vi "_reorder tool entries.vi"(11 "Path Control":path[](array[path])) -> (2 "After":string[](array[string]), 3 "Path Control (dup)":path[](array[path]))   [LabVIEW 2017, in "CSM DebugTool Dialog.lvlib"]
uses:
  CSM DebugTool Dialog.lvlib
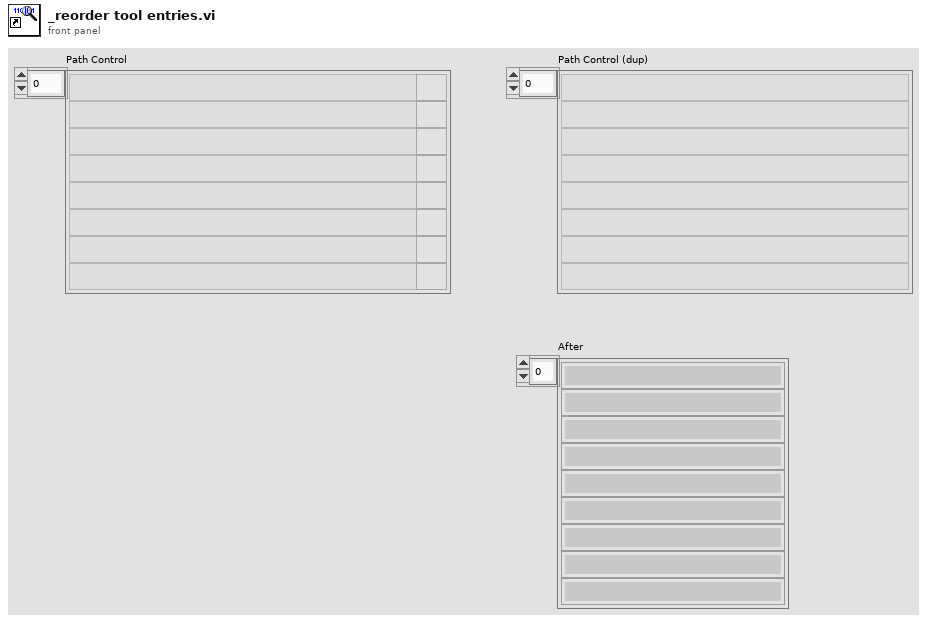
[diagram p1: front panel]
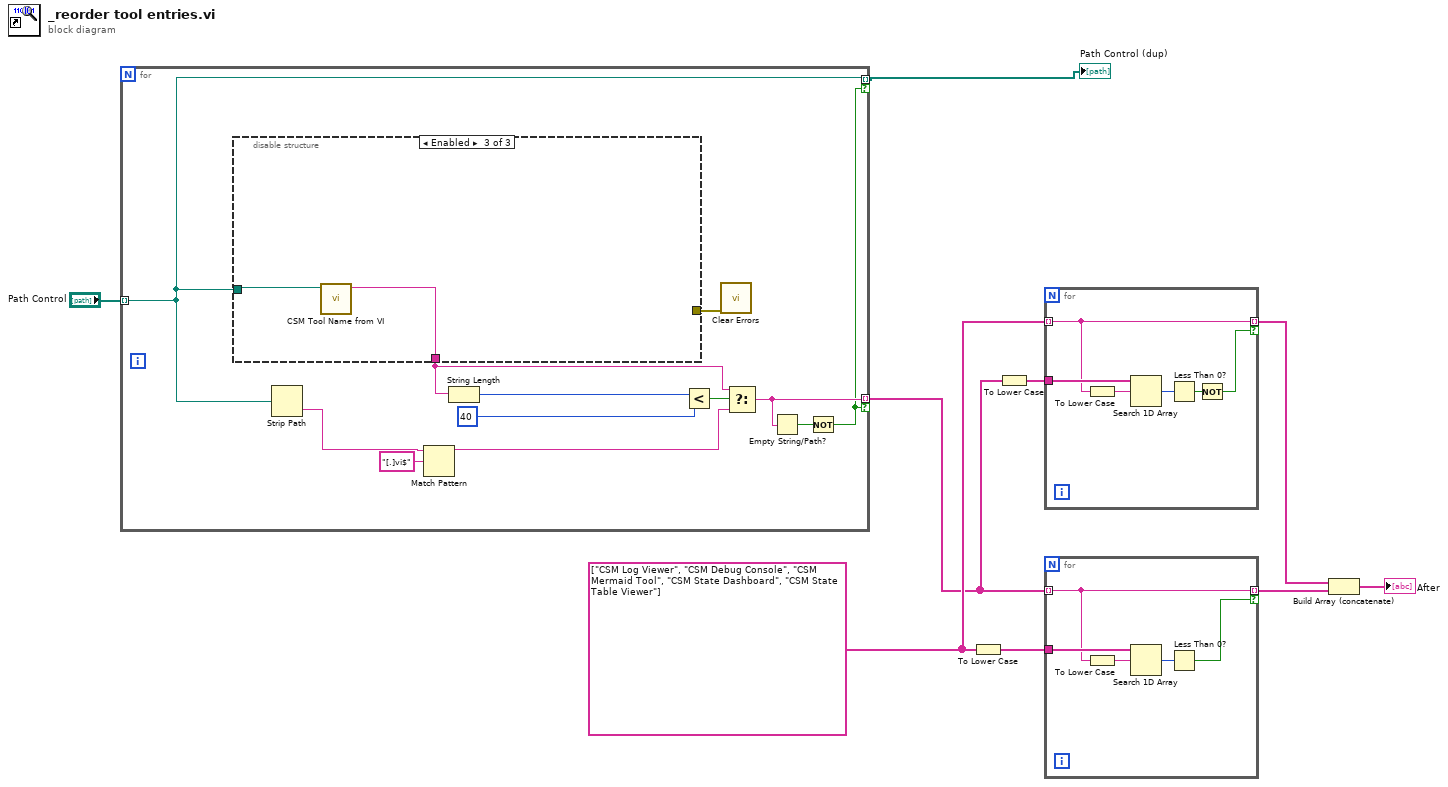
[diagram p0: block diagram]
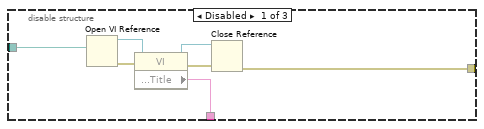
[diagram p2: hidden frame]
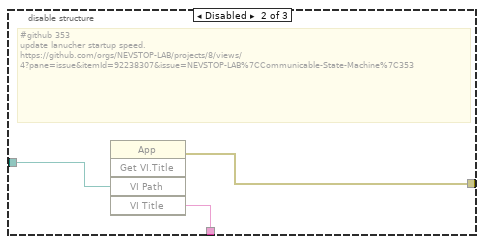
[diagram p3: hidden frame]
diagram:
  w6 = string[] ["CSM Log Viewer", "CSM Debug Console", "CSM Mermaid Tool", "CSM State Dashboard", "CSM State Table Viewer"] ("Before 2")
  n1 = for {
    tunnel: "Path Control" -> [w13] mode=indexing
    tunnel: [w12] -> w2 mode=indexing if=w10
    tunnel: [w13] -> w1 mode=indexing if=w10
    n2 = disable-structure shown="Enabled" {
      disable-tunnel: [w24 w29 _] -> w21
      disable-tunnel: w13 -> [w23 w31 w33]
      disable-tunnel: [w22 w30 w32] -> w19
      frame Disabled {
        n3 = Open VI Reference(vi path=w23) -> (vi reference=w28:refnum<vi>, error out=w27:errorcluster)  [unwired: 5 in]
        n4 = property class="VI"(reference=w28, error in=w27) -> (reference out=w25:refnum<vi>, error out=w26:errorcluster, "Front Panel.Title"=w22:string)
        n5 = Close Reference(reference=w25, error in (no error)=w26) -> (error out=w24:errorcluster)
      }
      frame Disabled {
        # "#github 353\nupdate lanucher startup speed.\nhttps://github.com/orgs/NEVSTOP-LAB/projects/8/views/4?pane=issue&itemId=92238307&issue=NEVSTOP-LAB%7CCommunicable-State-Machine%7C353"
        n6 = invoke class="App" method="Get VI.Title"("VI Path"=w31) -> (error out=w29:errorcluster, "VI Title"=w30:string)  [unwired: 4 in, 3 out]
      }
      frame Enabled {
        n7 = call "CSM Tool Name from VI.vi"("VI Path"=w33) -> ("ToolName"=w32:string)  [unwired: 10 in]
      }
    }
    n8 = Strip Path(path=w13) -> (name=w18:string)  [unwired: 1 out]
    n9 = Match Pattern(string=w18, regular expression="[.]vi$") -> (before substring=w16:string)  [unwired: 1 in, 3 out]
    n10 = String Length(string=w19) -> (length=w15:i32)
    n11 = Less?(x=w15, y=40) -> (x < y?=w20:bool)
    n12 = call <vilib>:"Clear Errors.vi"("error in (no error)"=w21) -> ()  [unwired: 5 in, 2 out]
    n13 = Select(t=w19, s=w20, f=w16) -> (s? t:f=w12:string)
    n14 = Empty String/Path?(string/path=w12) -> (empty?=w11:bool)
    n15 = Not(x=w11) -> (.not. x?=w10:bool)
  }
  "Path Control (dup)" <- w1
  n16 = To Lower Case(string=w6) -> (all lower case string=w8:string[])
  n17 = To Lower Case(string=w2) -> (all lower case string=w4:string[])
  n18 = for {
    tunnel: [w38] -> w5 mode=indexing if=w34
    tunnel: w6 -> [w38] mode=indexing
    tunnel: w4 -> [w39]
    n19 = To Lower Case(string=w38) -> (all lower case string=w37:string)
    n20 = Search 1D Array(1D array=w39, element=w37) -> (index of element=w36:i32)  [unwired: 1 in]
    n21 = Less Than 0?(x=w36) -> (x < 0?=w35:bool)
    n22 = Not(x=w35) -> (.not. x?=w34:bool)
  }
  n23 = for {
    tunnel: [w43] -> w9 mode=indexing if=w40
    tunnel: w2 -> [w43] mode=indexing
    tunnel: w8 -> [w44]
    n24 = To Lower Case(string=w43) -> (all lower case string=w42:string)
    n25 = Search 1D Array(1D array=w44, element=w42) -> (index of element=w41:i32)  [unwired: 1 in]
    n26 = Less Than 0?(x=w41) -> (x < 0?=w40:bool)
  }
  n27 = Build Array (concatenate)(w5, w9) -> (→"After":string[])
